vi "_GetLineLength.vi"(11 "Line":T1) -> (3 "Length":dbl)   [LabVIEW 2020, in "OpenLvVision_Overlays.lvlib"]
uses:
  TypeDefs/Line.ctl
  TypeDefs/PointI32.ctl
  OpenLvVision_Overlays.lvlib
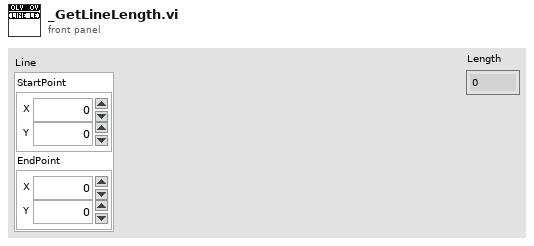
[diagram p1: front panel]
types:
  T1 = typedef "OpenLvVision_Overlays.lvlib/Line.ctl" = cluster{"StartPoint":T2, "EndPoint":T2}
  T2 = typedef "OpenLvVision_Overlays.lvlib/PointI32.ctl" = cluster{"X":i32, "Y":i32}
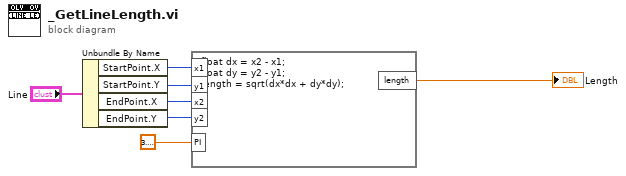
[diagram p0: block diagram]
diagram:
  n1 = Unbundle By Name("Line") -> ("StartPoint.X"=w5:i32, "StartPoint.Y"=w4:i32, "EndPoint.X"=w3:i32, "EndPoint.Y"=w2:i32)
  n2 = formula code="float dx = x2 - x1;\nfloat dy = y2 - y1;\nlength = sqrt(dx*dx + dy*dy);"("x1"=w5, "y1"=w4, "x2"=w3, "y2"=w2, "PI"=3.141592653589793) -> ("length"=→"Length":dbl)
